vi "RFH-add-Impedance_data.vi"() -> ()   [LabVIEW 2020, in "RFH-Reflection_File_Handler.lvlib"]
doc: "Run by hand: reads the files of a folder, computes the impedance with RDC-Lin-Calc_Impedance2 and saves them as common-format files. The user picks the folder and optionally a frequency template."
uses:
  RFH-Reflection_File_Handler.lvlib
  RFH-common_data_format.ctl
  Computation/RDC-Reflection_Data_Computation.lvlib
panel:
  in  "Use template?":bool
  in  "Clean up others":bool
  in  "X template":path=path "C:/projects/Universitet/Master/data/Ideal data/pb1-water1 M1.s2p"
  out "Data":T1
  out "converted file path":path
  out "error out":errorcluster
  in  "error in (no error)":errorcluster
  in  "folder path":path
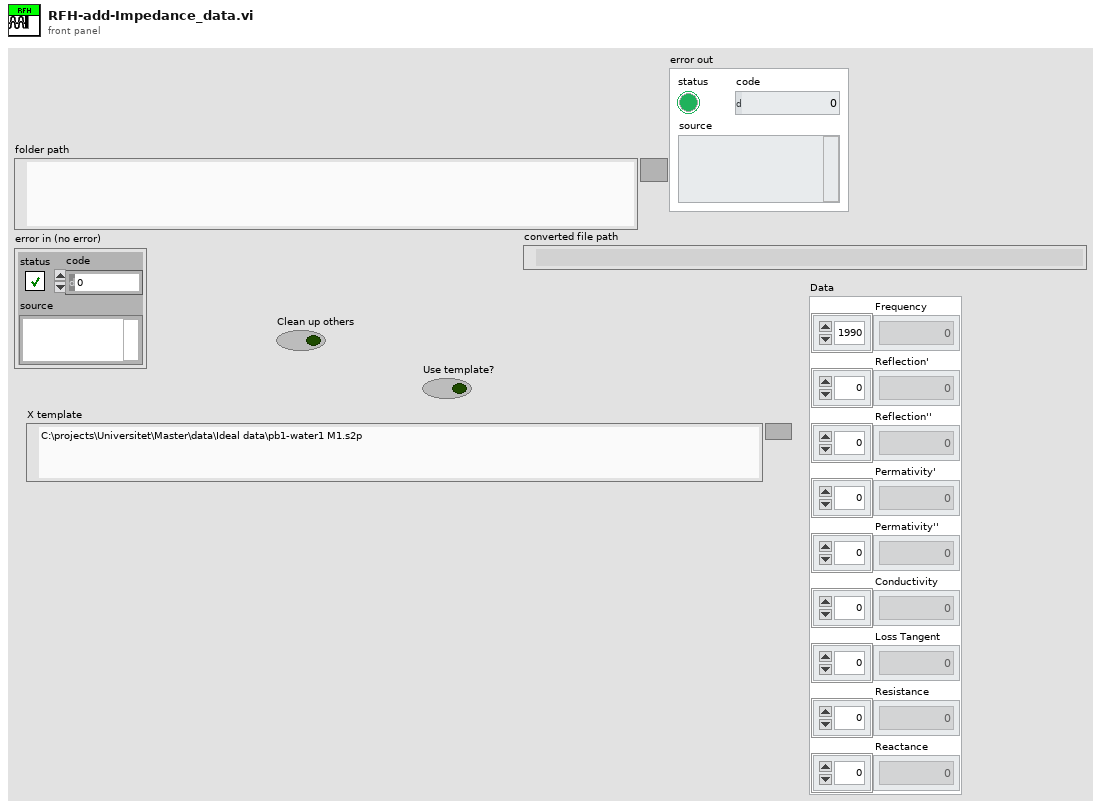
[diagram p1: front panel]
types:
  T1 = typedef "RFH-Reflection_File_Handler.lvlib/RFH-common_data_format.ctl" = cluster{"Frequency":dbl[], "Reflection'":dbl[], "Reflection''":dbl[], "Permativity'":dbl[], "Permativity''":dbl[], "Conductivity":dbl[], "Loss Tangent":dbl[], "Resistance":dbl[], "Reactance":dbl[]}
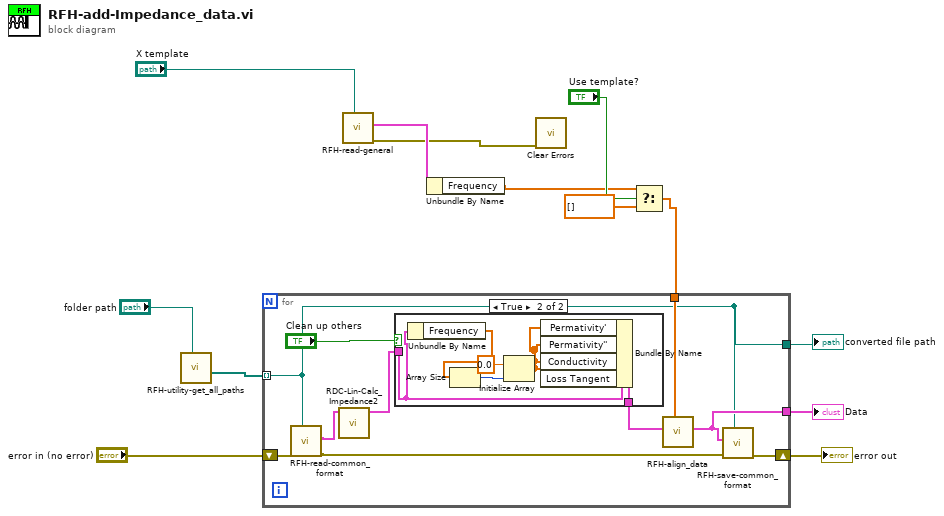
[diagram p0: block diagram]
diagram:
  n1 = call "RFH-utility-get_all_paths.vi"("Folder Path"="folder path") -> ("All Files in Dir"=w8:path[])  [unwired: 7 in, 3 out]
  n2 = call "RFH-read-general.vi"("file path (dialog if empty)"="X template") -> ("error out"=w5:errorcluster, "Common Format"=w6:T1)  [unwired: 9 in]
  n3 = Unbundle By Name(w6) -> ("Frequency"=w2:dbl[])
  n4 = call <vilib>:"Clear Errors.vi"("error in (no error)"=w5) -> ()  [unwired: 5 in, 2 out]
  n5 = Select(t=w2, s="Use template?", f=dbl[] []) -> (s? t:f=w1:dbl[])
  n6 = for {
    tunnel: w1 -> [w22]
    tunnel: [w21] -> w10
    shift-right: [w23] -> w12
    shift-left: "error in (no error)" -> [w20]
    tunnel: w8 -> [w19] mode=indexing
    tunnel: [w19] -> w13
    n7 = call "RFH-read-common_format.vi"("file path (dialog if empty)"=w19, "error in"=w20) -> ("error out"=w17:errorcluster, "Common Format"=w18:T1)  [unwired: 8 in]
    n8 = call "RDC-Lin-Calc_Impedance2.vi"("input cluster"=w18) -> ("Output cluster"=w15:T1)  [unwired: 9 in, 1 out]
    n9 = case shown="True" "Clean up others" {
      tunnel: [w24 w30] -> w16
      tunnel: w15 -> [w24 w29]
      frame False {
      }
      frame True {
        n10 = Unbundle By Name(w29) -> ("Frequency"=w28:dbl[])
        n11 = Array Size(array=w28) -> (size(s)=w27:i32)
        n12 = Initialize Array(0.0 ("element"), w27) -> (w25:dbl[])
        n13 = Bundle By Name(cluster=w29, "Permativity'"=w25, "Permativity''"=w25, "Conductivity"=w25, "Loss Tangent"=w25) -> (w30:T1)
      }
    }
    n14 = call "RFH-align_data.vi"("Xi"=w22, "Common Format"=w16) -> ("Common Format alligned"=w21:T1)  [unwired: 9 in]
    n15 = call "RFH-save-common_format.vi"("file path (use dialog)"=w19, "error in (no error)"=w17, "Common Format"=w21) -> ("error out"=w23:errorcluster)  [unwired: 8 in]
  }
  "error out" <- w12
  "converted file path" <- w13
  "Data" <- w10
